vi "User Authentication Schemes.vi"(5 "Username":string, 7 "Address":string, 8 "Error In":errorcluster) -> (0 "Error Out":errorcluster)   [LabVIEW 2018, in "Tests.lvlib" / "Session.lvlib"]
uses:
  Session.lvlib
  src/Toolkit/Session/Type Definitions/User Authentication Schemes.ctl
  src/Toolkit/Session/Support/Create from SSH.vi
  src/Toolkit/Session/Support/Destroy to SSH.vi
  <vilib>/addons/_JKI Toolkits/Caraya/classes/Test/Test.lvclass
  src/Toolkit/SSH/SSH.lvclass
  src/Toolkit/Session/Session.lvclass
  <vilib>/addons/_JKI Toolkits/Caraya/classes/Assert/Assert.lvclass
  Tests.lvlib
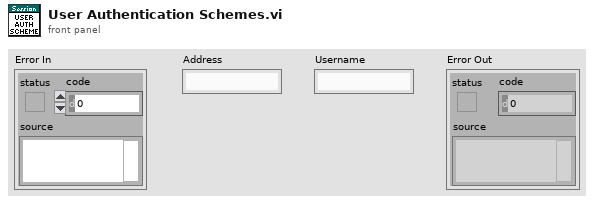
[diagram p1: front panel]
types:
  T1 = typedef "Toolkit.lvlib/Session.lvclass/User Authentication Schemes.ctl" = enum16{"Keyboard", "Password", "Public Key"}
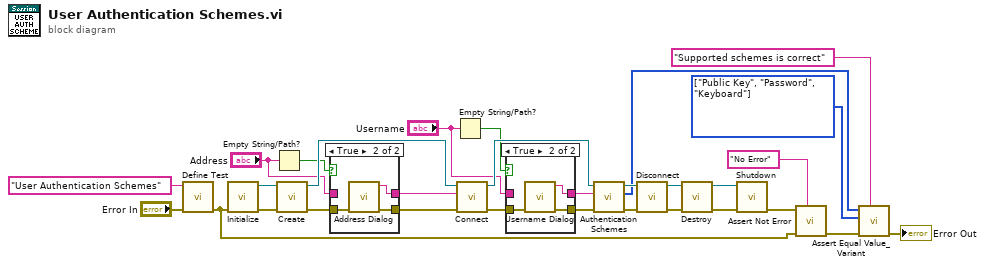
[diagram p0: block diagram]
diagram:
  w11 = T1[] [enum."Public Key", enum."Password", enum."Keyboard"] items=["Keyboard", "Password", "Public Key"] ("Supported Schemes")
  n1 = call <vilib>:"Define Test.vi"("error in (no error)"="Error In", "Label (VI Title)"="User Authentication Schemes") -> ("error out"=w22:errorcluster)  [unwired: 9 in]
  n2 = call "Initialize.vi"("Error In"=w22) -> ("Error Out"=w28:errorcluster, "SSH"=w27:refnum<class "SSH.lvclass">)  [unwired: 9 in]
  n3 = Empty String/Path?(string/path="Address") -> (empty?=w7:bool)
  n4 = call-poly "Create.vi"("Error In"=w28, "SSH"=w27) -> ("Error Out"=w5:errorcluster, "Sesssion"=w21:refnum<class "Session.lvclass">)  [unwired: 8 in]
  n5 = case shown="True" w7 {
    tunnel: w5 -> [w31 w35]
    tunnel: [w31 w34] -> w3
    tunnel: [w32 w33] -> w4
    tunnel: "Address" -> [w32 _]
    frame False {
    }
    frame True {
      n6 = call "Address Dialog.vi"("Error In"=w35) -> ("Error Out"=w34:errorcluster, "Address Out"=w33:string)  [unwired: 9 in]
    }
  }
  n7 = Empty String/Path?(string/path="Username") -> (empty?=w2:bool)
  n8 = call "Connect.vi"("Error In"=w3, "Address"=w4, "Session In"=w21) -> ("Error Out"=w10:errorcluster, "Sesssion Out"=w18:refnum<class "Session.lvclass">)  [unwired: 7 in]
  n9 = case shown="True" w2 {
    tunnel: w10 -> [w36 w40]
    tunnel: [w36 w39] -> w9
    tunnel: [w37 w38] -> w8
    tunnel: "Username" -> [w37 _]
    frame False {
    }
    frame True {
      n10 = call "Username Dialog.vi"("Error In"=w40) -> ("Error Out"=w39:errorcluster, "Username Out"=w38:string)  [unwired: 9 in]
    }
  }
  n11 = call "Authentication Schemes.vi"("Error In"=w9, "Username"=w8, "Session In"=w18) -> ("Error Out"=w16:errorcluster, "Supported Schemes"=w12:T1[], "Sesssion Out"=w17:refnum<class "Session.lvclass">)  [unwired: 6 in]
  n12 = call "Disconnect.vi"("Error In"=w16, "Session In"=w17) -> ("Error Out"=w19:errorcluster, "Sesssion Out"=w20:refnum<class "Session.lvclass">)  [unwired: 8 in]
  n13 = call-poly "Destroy.vi"("Error In"=w19, "Session"=w20) -> ("Error Out"=w25:errorcluster, "SSH"=w26:refnum<class "SSH.lvclass">)  [unwired: 8 in]
  n14 = call "Shutdown.vi"("Error In"=w25, "SSH"=w26) -> ("Error Out"=w24:errorcluster)  [unwired: 9 in]
  n15 = call <vilib>:"Assert Not Error.vi"("Label"="No Error", "error in (no error)"=w22, "Not Error?"=w24) -> ("error out"=w15:errorcluster)  [unwired: 8 in]
  n16 = call <vilib>:"Assert Equal Value_Variant.vi"("Label"="Supported schemes is correct", "error in (no error)"=w15, "Y"=w11, "X"=w12) -> ("error out"=→"Error Out":errorcluster)  [unwired: 7 in]
